vi "Name of Build Specification--constant.vi"() -> (3 "Name of Build Specification":string)   [LabVIEW 2026]
doc: "This constant represents the name of the build specification for the modules PPL in the template project."
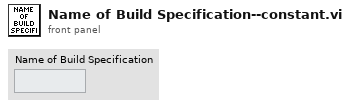
[diagram p1: front panel]
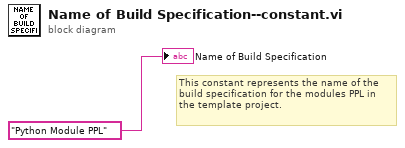
[diagram p0: block diagram]
diagram:
  # "This constant represents the name of the build specification for the modules PPL in the template project."
  "Name of Build Specification" <- "Python Module PPL" ("Name of Build Specification")
